vi "Log Error.vi"(8 "error in (no error)":errorcluster, 10 "Message":string, 11 "Logging In":refnum<class "Logging.lvclass">) -> (0 "error out":errorcluster, 3 "Logging Out":refnum<class "Logging.lvclass">)   [LabVIEW 2020, in "Logging.lvclass"]
doc: "Enter an error-level message into the system log.\nAn error occurs due to a more serious problem, the software has not been able to perform some function.\nLogging is not meant as a substitute for error handling."
uses:
  Logging.lvclass
  Protected/Level.ctl
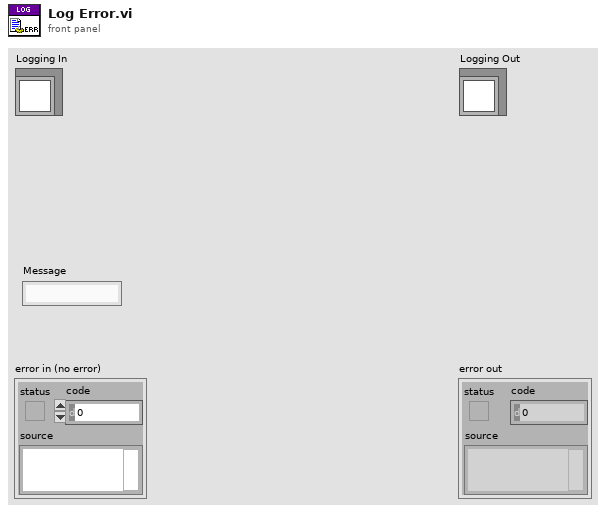
[diagram p1: front panel]
types:
  T1 = typedef "Logging.lvclass/Level.ctl" = enum16{"DEBUG", "INFO", "WARNING", "ERROR", "CRITICAL"}
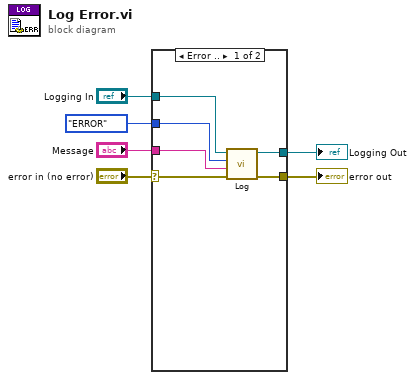
[diagram p0: block diagram]
diagram:
  n1 = case shown="Error .." "error in (no error)" {
    selector: "error in (no error)" -> [w8 w13]
    tunnel: [w12 w13] -> w6
    tunnel: "Logging In" -> [w11 w14]
    tunnel: [w10 w14] -> w4
    tunnel: Level."ERROR" ("Level") -> [w9 _]
    tunnel: "Message" -> [w7 _]
    frame Error {
      n2 = call-dynamic "Log.vi"("error in (no error)"=w8, "Message"=w7, "Level"=w9, "Logging In"=w11) -> ("error out"=w12:errorcluster, "Logging Out"=w10:refnum<class "Logging.lvclass">)  [unwired: 6 in]
    }
    frame No Error {
    }
  }
  "error out" <- w6
  "Logging Out" <- w4
